vi "Format Tree.vi"(9 "Update":bool, 10 "Commands":cluster{"Time (s)":dbl, T1, bool}[](array[cluster]), 11 "Tree Refnum":refnum<vi>) -> ()   [LabVIEW 2023]
uses:
  Types/Single Cmd Info.ctl
  <vilib>/picture/picture.llb/imagedata.ctl
  <vilib>/Utility/Data Type/NI_Data Type.lvlib
panel:
  in  "Tree":string(tree)
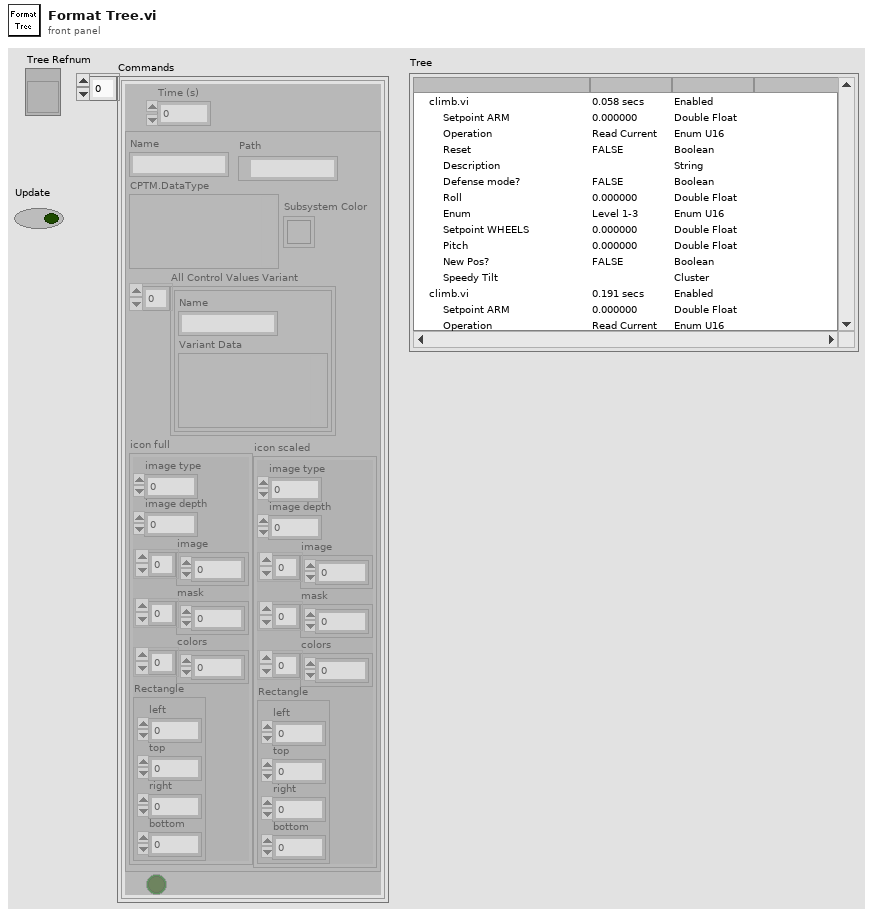
[diagram p1: front panel]
types:
  T1 = typedef "Single Cmd Info.ctl" = cluster{"Name":string, "CPTM.DataType":variant, "All Control Values Variant":cluster{"Name":string, "Variant Data":variant}[], "icon full":T2, "icon scaled":T2, "Path":path, "Subsystem Color":u32}
  T2 = typedef "imagedata.ctl" = cluster{"image type":i32, "image depth":i32, "image":u8[], "mask":u8[], "colors":u32[], "Rectangle":cluster{"left":i16, "top":i16, "right":i16, "bottom":i16}}
  T3 = cluster{"Left Cell String":string, "Child Text":string[], "Child Tag":string, "Item Indent":i32, "Child Only?":bool, "Glyph Index":i32}
  T4 = cluster{"Left Cell String":string, "Child Text":string[], "Child Tag":string, "Item Indent":i32, "Child Only?":bool, "Glyph Index":i32}[]
  T5 = typedef "NI_Data Type.lvlib/Data Type.ctl" = enum8{"Invalid Type", "Void", "I8", "I16", "I32", "I64", "U8", "U16", "U32", "U64", "Single Float", "Double Float", "Extended Float", "Single Complex", "Double Complex", "Extended Complex", "Enum U8", "Enum U16", "Enum U32", "Enum U64", "Single Float With Unit", "Double Float With Unit", "Extended Float With Unit", "Single Complex with Unit", "Double Complex with Unit", "Extended Complex with Unit", "Boolean", "String", "Path", "Picture", "Tag", "Array", "Cluster", "Variant", "LV Variant", "Waveform", "Timestamp", "Digital Waveform", "Digital Data", "ExpressData", "Refnum", "External Data", "VI", "Poly VI", "LabVIEW Class Instance", "Fixed Point", "Set Collection", "Map Collection"}
  T6 = typedef "NI_Data Type.lvlib/Type Definition Info.ctl" = cluster{"Name":string, "Timestamp":u32}
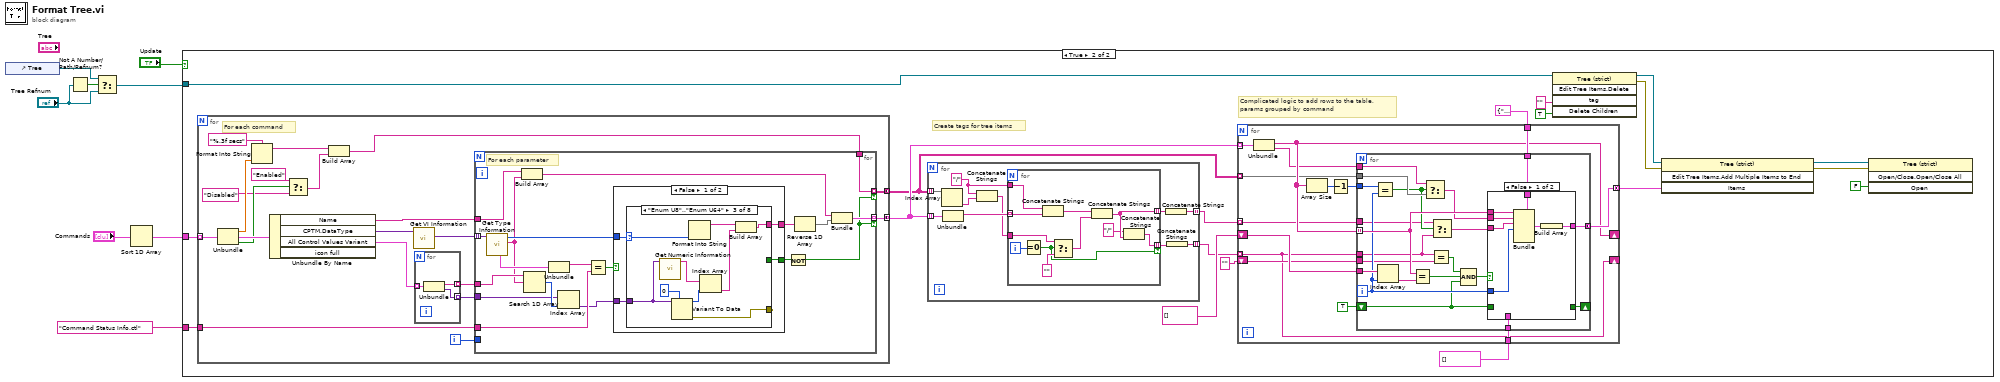
[diagram p0: block diagram]
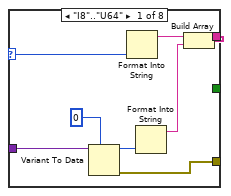
[diagram p4: hidden frame]
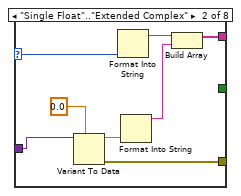
[diagram p5: hidden frame]
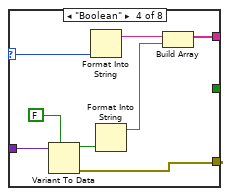
[diagram p6: hidden frame]
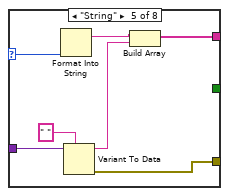
[diagram p7: hidden frame]
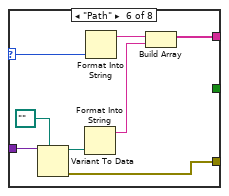
[diagram p8: hidden frame]
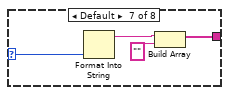
[diagram p9: hidden frame]
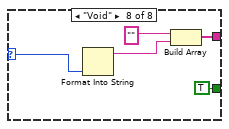
[diagram p10: hidden frame]
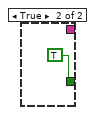
[diagram p11: hidden frame]
diagram:
  n1 = control-ref of="Tree"() -> (w6:refnum<vi>)
  n2 = Not A Number/Path/Refnum?(number/path/refnum="Tree Refnum") -> (NaN/Path/Refnum?=w8:bool)
  n3 = Select(t=w6, s=w8, f="Tree Refnum") -> (s? t:f=w3:refnum<vi>)
  n4 = Sort 1D Array(array="Commands") -> (sorted array=w2:cluster{"Time (s)":dbl, T1, bool}[])
  n5 = case shown="True" "Update" {
    tunnel: "Command Status Info.ctl" ("Name") -> [_ w27]
    tunnel: w3 -> [_ w14]
    tunnel: w2 -> [_ w13]
    frame False {
    }
    frame True {
      # "Complicated logic to add rows to the table,\nparams grouped by command"
      # "Create tags for tree items"
      n6 = for {
        tunnel: [w89] -> w12 mode=concatenating
        tunnel: w27 -> [w84]
        tunnel: w13 -> [w82] mode=indexing
        tunnel: [w73] -> w11 mode=concatenating
        i -> [w85]
        # "For each command"
        n7 = Unbundle(w82) -> ("Time (s)"=w80:dbl, w83:T1, w79:bool)
        n8 = Format Into String(format string="%.3f secs", w80) -> (resulting string=w76:string)  [unwired: 2 in, 1 out]
        n9 = Unbundle By Name(w83) -> ("Name"=w81:string, "CPTM.DataType"=w91:variant, "All Control Values Variant"=w88:cluster{"Name":string, "Variant Data":variant}[])  [unwired: 1 out]
        n10 = Select(t="Enabled", s=w79, f="Disabled") -> (s? t:f=w75:string)
        n11 = Build Array(w76, w75) -> (w74:string[])
        n12 = call <vilib>:"Get VI Information.vi"("variant"=w91) -> ("VI terminal types"=w90:variant[])  [unwired: 7 in, 3 out]
        n13 = for {
          tunnel: w88 -> [w175] mode=indexing
          tunnel: [w174] -> w87 mode=indexing
          tunnel: [w173] -> w86 mode=indexing
          n14 = Unbundle(w175) -> ("Name"=w174:string, "Variant Data"=w173:variant)
        }
        n15 = for {
          tunnel: w90 -> [w110] mode=indexing
          tunnel: [w107] -> w89 mode=indexing if=w92
          tunnel: w84 -> [w105]
          tunnel: w87 -> [w100]
          tunnel: w86 -> [w97]
          tunnel: w85 -> [_]
          tunnel: w81 -> [w95]
          tunnel: w74 -> [w93]
          tunnel: [w93] -> w73 mode=indexing if=w92
          # "For each parameter"
          n16 = call <vilib>:"Get Type Information.vi"("variant"=w110) -> ("name"=w99:string, "type"=w109:T5, "type definition info"=w106:T6)  [unwired: 6 in, 2 out]
          n17 = Build Array(w95, w99) -> (w108:string[])
          n18 = Search 1D Array(1D array=w100, element=w99) -> (index of element=w98:i32)  [unwired: 1 in]
          n19 = Unbundle(w106) -> ("Name"=w104:string)  [unwired: 1 out]
          n20 = Index Array(array=w97, index=w98) -> (element=w96:variant)
          n21 = Equal?(x=w104, y=w105) -> (x = y?=w103:bool)
          n22 = case shown="False" w103 {
            tunnel: w109 -> [w114 _]
            tunnel: [w113 _] -> w101
            tunnel: [w112 TRUE] -> w102
            tunnel: w96 -> [w111 _]
            frame False {
              n23 = case shown="\"Enum U8\"..\"Enum U64\"" w114 {
                selector: w114 -> [w122 w130 w139 w147 w154 w162 w166 w171]
                tunnel: [w117 w124 w136 w142 w151 w157 w164 w168] -> w113
                tunnel: [_ _ _ _ _ _ _ TRUE] -> w112
                tunnel: w111 -> [w116 w127 w134 w144 w153 w159 _ _]
                tunnel: [w115 w123 w135 w140 w148 w155 _ _] -> _
                frame "I8".."U64" {
                  n24 = Variant To Data(type=i64 0, Variant=w116) -> (data=w120:i64, error out=w115:errorcluster)  [unwired: 1 in]
                  n25 = Format Into String(w122) -> (resulting string=w118:string)  [unwired: 3 in, 1 out]
                  n26 = Format Into String(w120) -> (resulting string=w119:string)  [unwired: 3 in, 1 out]
                  n27 = Build Array(w118, w119) -> (w117:string[])
                }
                frame "Single Float".."Extended Complex" {
                  n28 = Variant To Data(type=0.0, Variant=w127) -> (data=w128:dbl, error out=w123:errorcluster)  [unwired: 1 in]
                  n29 = Format Into String(w130) -> (resulting string=w126:string)  [unwired: 3 in, 1 out]
                  n30 = Format Into String(w128) -> (resulting string=w125:string)  [unwired: 3 in, 1 out]
                  n31 = Build Array(w126, w125) -> (w124:string[])
                }
                frame "Enum U8".."Enum U64" {
                  n32 = call <vilib>:"Get Numeric Information.vi"("variant"=w134) -> ("enum names"=w133:string[])  [unwired: 7 in, 3 out]
                  n33 = Variant To Data(type=i64 0, Variant=w134) -> (data=w132:i64, error out=w135:errorcluster)  [unwired: 1 in]
                  n34 = Format Into String(w139) -> (resulting string=w137:string)  [unwired: 3 in, 1 out]
                  n35 = Index Array(array=w133, index=w132) -> (element=w131:string)
                  n36 = Build Array(w137, w131) -> (w136:string[])
                }
                frame "Boolean" {
                  n37 = Variant To Data(type=FALSE, Variant=w144) -> (data=w145:bool, error out=w140:errorcluster)  [unwired: 1 in]
                  n38 = Format Into String(w147) -> (resulting string=w143:string)  [unwired: 3 in, 1 out]
                  n39 = Format Into String(w145) -> (resulting string=w141:string)  [unwired: 3 in, 1 out]
                  n40 = Build Array(w143, w141) -> (w142:string[])
                }
                frame "String" {
                  n41 = Format Into String(w154) -> (resulting string=w152:string)  [unwired: 3 in, 1 out]
                  n42 = Variant To Data(type=" ", Variant=w153) -> (data=w150:string, error out=w148:errorcluster)  [unwired: 1 in]
                  n43 = Build Array(w152, w150) -> (w151:string[])
                }
                frame "Path" {
                  n44 = Variant To Data(type=path "", Variant=w159) -> (data=w160:path, error out=w155:errorcluster)  [unwired: 1 in]
                  n45 = Format Into String(w160) -> (resulting string=w156:string)  [unwired: 3 in, 1 out]
                  n46 = Format Into String(w162) -> (resulting string=w158:string)  [unwired: 3 in, 1 out]
                  n47 = Build Array(w158, w156) -> (w157:string[])
                }
                frame Default {
                  n48 = Format Into String(w166) -> (resulting string=w165:string)  [unwired: 3 in, 1 out]
                  n49 = Build Array(w165, "") -> (w164:string[])
                }
                frame "Void" {
                  n50 = Format Into String(w171) -> (resulting string=w169:string)  [unwired: 3 in, 1 out]
                  n51 = Build Array("", w169) -> (w168:string[])
                }
              }
            }
            frame True {
            }
          }
          n52 = Not(x=w102) -> (.not. x?=w92:bool)
          n53 = Reverse 1D Array(array=w101) -> (reversed array=w94:string[])
          n54 = Bundle(w108, w94) -> (w107:cluster{string[], string[]})  [unwired: 1 in]
        }
      }
      n55 = for {
        tunnel: w12 -> [w185] mode=indexing
        tunnel: [w182] -> w24 mode=indexing
        tunnel: w11 -> [w181] mode=indexing
        tunnel: [w177] -> w10 mode=indexing
        w176 = "/"
        n56 = Index Array(array=w181) -> (element=w180:string)  [unwired: 1 in]
        n57 = Unbundle(w185) -> (w184:string[])  [unwired: 1 out]
        n58 = Concatenate Strings(w176, w180) -> (w179:string)
        n59 = for {
          tunnel: w184 -> [w196] mode=indexing
          tunnel: [w189] -> w183 mode=indexing
          tunnel: w179 -> [w192]
          tunnel: [w188] -> w178 mode=indexing if=w190
          tunnel: w176 -> [w186]
          i -> [w195]
          n60 = Equal To 0?(x=w195) -> (x = 0?=w190:bool)
          n61 = Concatenate Strings(w186, w196) -> (w194:string)
          n62 = Select(t=w192, s=w190, f="") -> (s? t:f=w191:string)
          n63 = Concatenate Strings(w194, w191) -> (w189:string)
          n64 = Concatenate Strings("/", w189) -> (w188:string)
        }
        n65 = Concatenate Strings(w183) -> (w182:string)
        n66 = Concatenate Strings(w178) -> (w177:string)
      }
      n67 = for {
        tunnel: [w37] -> w15 mode=concatenating
        tunnel: T3 {"Left Cell String"="", "Child Text"=[], "Child Tag"="", "Item Indent"=0, "Child Only?"=FALSE, "Glyph Index"=0} ("Item") -> [w38]
        shift-right: [w34] -> _
        shift-left: string[] [] ("Child Text") -> [w40]
        tunnel: w12 -> [w41] mode=indexing
        tunnel: T4 [] -> [w39]
        tunnel: w24 -> [w33] mode=indexing
        tunnel: w11 -> [w30] mode=indexing
        tunnel: w10 -> [w28] mode=indexing
        shift-right: [w28] -> _
        shift-left: "" -> [w29]
        n68 = Unbundle(w41) -> (w34:string[], w31:string[])
        n69 = Array Size(array=w34) -> (size(s)=w36:i32)
        n70 = Decrement(x=w36) -> (x-1=w35:i32)
        n71 = for {
          tunnel: w40 -> [w62]
          tunnel: w34 -> [w57] mode=indexing
          tunnel: w39 -> [w60]
          tunnel: [w59] -> w37 mode=concatenating
          tunnel: w38 -> [w58]
          tunnel: w35 -> [w55]
          tunnel: w31 -> [w49]
          tunnel: w33 -> [w45]
          shift-right: [w52] -> _
          shift-left: TRUE -> [w51]
          tunnel: w30 -> [w48]
          tunnel: w28 -> [w44]
          tunnel: w29 -> [w43]
          i -> [w56]
          n72 = Equal?(x=w55, y=w56) -> (x = y?=w47:bool)
          n73 = Index Array(array=w62, index=w56) -> (element=w61:string)
          n74 = Equal?(x=w57, y=w61) -> (x = y?=w54:bool)
          n75 = Select(t=w49, s=w47, f=w48) -> (s? t:f=w50:string[])
          n76 = Equal?(x=w44, y=w43) -> (x = y?=w42:bool)
          n77 = Select(t=w45, s=w47, f=w44) -> (s? t:f=w46:string)
          n78 = Compound Arithmetic op=AND(w42, w54, w51) -> (w53:bool)
          n79 = case shown="False" w53 {
            tunnel: [w67 w71] -> w59
            tunnel: w60 -> [_ w71]
            tunnel: w58 -> [w69 _]
            tunnel: w57 -> [w66 _]
            tunnel: w56 -> [w65 _]
            tunnel: w50 -> [w64 _]
            tunnel: w46 -> [w63 _]
            tunnel: [_ w70] -> w52
            tunnel: w51 -> [_ w70]
            frame False {
              n80 = Bundle(cluster=w69, "Left Cell String"=w66, "Child Text"=w64, "Child Tag"=w63, "Item Indent"=w65) -> (w68:T3)  [unwired: 2 in]
              n81 = Build Array(w68) -> (w67:T4)
            }
            frame True {
            }
          }
        }
      }
      n82 = invoke on="Invoke Node" class="Tree (strict)" method="Edit Tree Items.Delete"(reference=w14, "tag"="" ("Tag"), "Delete Children"=TRUE ("Delete Children?")) -> (reference out=w21:refnum<vi>, error out=w16:errorcluster)  [unwired: 2 in, 3 out]
      n83 = invoke on="Invoke Node" class="Tree (strict)" method="Edit Tree Items.Add Multiple Items to End"(reference=w21, error in=w16, "Items"=w15) -> (reference out=w22:refnum<vi>, error out=w19:errorcluster)  [unwired: 1 in, 2 out]
      n84 = invoke on="Invoke Node" class="Tree (strict)" method="Open/Close.Open/Close All"(reference=w22, error in=w19, "Open"=FALSE ("Open?")) -> ()  [unwired: 1 in, 4 out]
    }
  }
